vi "Load Config.vi"(8 "error in (no error)":errorcluster, 11 "VolatusConfig in":refnum<class "VolatusConfig.lvclass">) -> (0 "error out":errorcluster, 3 "VolatusConfig out":refnum<class "VolatusConfig.lvclass">, 5 "Config Path":path)   [LabVIEW 2020, in "VolatusConfig.lvlib" / "VolatusConfig.lvclass"]
uses:
  VolatusConfig.lvclass
  lv-web-crypto/lv-crypto/Crypto/Hashes/SHA-256/SHA-256.lvclass
  VolatusConfig.lvclass/VolatusConfig.ctl
  lv-cdm/CDM-Config/Config Storage/Config Storage.lvclass
  lv-web-crypto/lv-crypto/Crypto/Crypto.lvlib
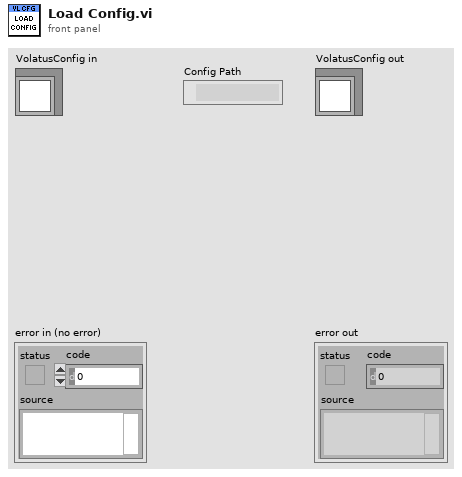
[diagram p1: front panel]
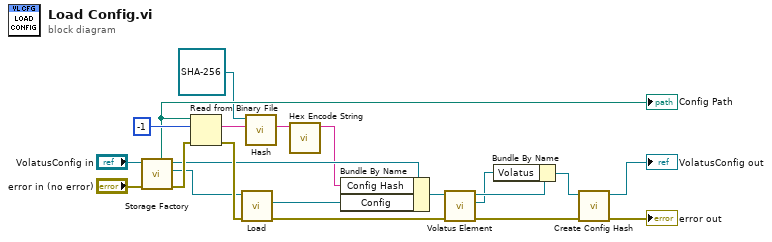
[diagram p0: block diagram]
diagram:
  n1 = call "Storage Factory.vi"("error in (no error)"="error in (no error)", "VolatusConfig in"="VolatusConfig in") -> ("error out"=w21:errorcluster, "Storage"=w16:refnum<class "Config Storage.lvclass">, "VolatusConfig out"=w17:refnum<class "VolatusConfig.lvclass">, "Config Path"=w13:path)  [unwired: 6 in]
  "Config Path" <- w13
  n2 = Read from Binary File(8:w21, 10:-1 ("count (1)"), 11:w13) -> (0:w20:errorcluster, 2:w6:string)  [unwired: 3 in, 2 out]
  n3 = call "Load.vi"("error in (no error)"=w20, "Config Storage in"=w16) -> ("error out"=w2:errorcluster, "Config"=w15:refnum<class "Config Manager.lvclass">)  [unwired: 7 in, 1 out]
  n4 = call-dynamic "Hash.vi"("Message"=w6, "SHA-256 in"=refnum<class "SHA-256.lvclass"> refnum ("Crypto.lvlib:SHA-256.lvclass")) -> ("Hash"=w4:string)  [unwired: 7 in, 2 out]
  n5 = call "Hex Encode String.vi"("String"=w4) -> ("Hex Encoded String"=w3:string)  [unwired: 10 in]
  n6 = Bundle By Name(cluster=w17, "Config Hash"=w3, "Config"=w15) -> (w11:refnum<class "VolatusConfig.lvclass">)
  n7 = call "Volatus Element.vi"("error in (no error)"=w2, "VolatusConfig in"=w11) -> ("error out"=w1:errorcluster, "Volatus Element"=w7:refnum<class "Config Element.lvclass">, "VolatusConfig out"=w9:refnum<class "VolatusConfig.lvclass">)  [unwired: 7 in]
  n8 = Bundle By Name(cluster=w9, "Volatus"=w7) -> (w8:refnum<class "VolatusConfig.lvclass">)
  n9 = call "Create Config Hash.vi"("error in (no error)"=w1, "VolatusConfig in"=w8) -> ("error out"=→"error out":errorcluster, "VolatusConfig out"=→"VolatusConfig out":refnum<class "VolatusConfig.lvclass">)  [unwired: 8 in]
